vi "Scale List Write Item.vi"(8 "Scale Index":i32, 9 "r坐标轴列表":refnum<vi>, 10 "Sacle Setting":T1, 11 "Data Viewer in":refnum<class "Data Viewer.lvclass">) -> (3 "Data Viewer out":refnum<class "Data Viewer.lvclass">)   [LabVIEW 2020, in "Data Viewer.lvlib" / "Data Viewer.lvclass"]
uses:
  Data Viewer.lvclass
  Scale Setting--cluster.ctl
  Data Viewer.lvclass/Data Viewer.ctl
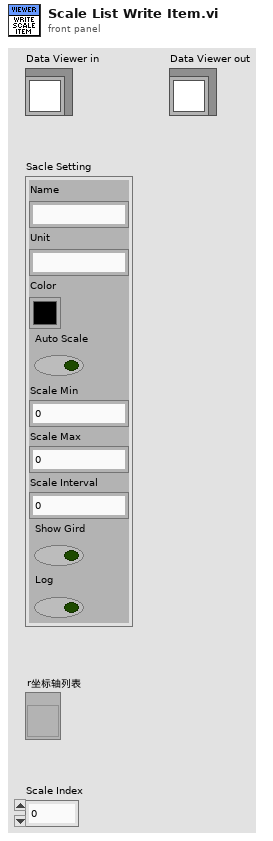
[diagram p1: front panel]
types:
  T1 = typedef "Data Viewer.lvlib/Data Viewer.lvclass/Scale Setting--cluster.ctl" = cluster{"Name":string, "Unit":string, "Color":u32, "Auto Scale":bool, "Scale Min":dbl, "Scale Max":dbl, "Scale Interval":dbl, "Show Gird":bool, "Log":bool}
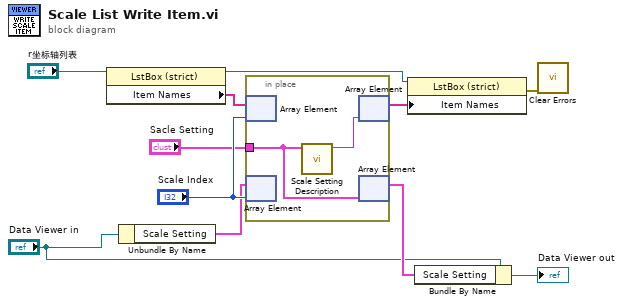
[diagram p0: block diagram]
diagram:
  n1 = property class="LstBox (strict)"(reference="r坐标轴列表") -> (reference out=w7:refnum<vi>, "Item Names"=w9:string[])  [unwired: 1 in, 1 out]
  n2 = Unbundle By Name("Data Viewer in") -> ("Scale Setting"=w2:T1[])
  n3 = in-place {
    in-place-border: "Sacle Setting" -> [w13]
    n4 = in-place-array #1(w9, "Scale Index") -> ()  [unwired: 1 out]
    n5 = in-place-array #2(w2, "Scale Index") -> ()  [unwired: 1 out]
    n6 = call "Scale Setting Description.vi"("Sacle Setting Out"=w13) -> ("Description"=w12:string)  [unwired: 10 in]
    n7 = in-place-array #1(w12) -> (w11:string[])  [unwired: 1 out]
    n8 = in-place-array #2(w13) -> (w6:T1[])  [unwired: 1 out]
  }
  n9 = property class="LstBox (strict)"(reference=w7, "Item Names"=w11) -> (error out=w8:errorcluster)  [unwired: 1 in, 1 out]
  n10 = Bundle By Name(cluster="Data Viewer in", "Scale Setting"=w6) -> (→"Data Viewer out":refnum<class "Data Viewer.lvclass">)
  n11 = call <vilib>:"Clear Errors.vi"("error in (no error)"=w8) -> ()  [unwired: 5 in, 2 out]
